vi "Turn.vi"(8 "Speed (0-30)":dbl=15.0, 11 "Angle (degrees)":i32=360) -> ()   [LabVIEW 2017]
uses:
  <vilib>/FPGAPlugInAG/myRIO-1900/niLvFpga_Open_myRIO-1900.vi
  <vilib>/rvi/interface/common/dynamic/niFpgaDynamicAddResources.vi
  <vilib>/Utility/error.llb/Error Cluster From Error Code.vi
  <vilib>/rvi/errors/niLvFpgaAdjustHostInterfaceError.vi
  <vilib>/FPGAPlugInAG/Dynamic/niLvFpga_Run_Dynamic.vi
  <vilib>/FPGAPlugInAG/Dynamic/niLvFpga_Close_Dynamic.vi
  <vilib>/rvi/interface/nirviOpenFPGA/nirviOpenFPGA.xnode
  FPGA Bitfiles/BadassLoader_FPGATarget_DCMotorControlle_4dRX-8eX8o0.lvbitx
  <vilib>/rvi/interface/nirviReadWriteControl/nirviReadWriteControl.xnode
  <vilib>/rvi/interface/nirviMethod/nirviMethod.xnode
  <vilib>/rvi/interface/nirviCloseFPGA/nirviCloseFPGA.xnode
  <vilib>/rvi/interface/Simulation/niFpgaSimulationCallBeginRW.vi
  NiFpgaLv.dll
panel:
  in  "stop":bool
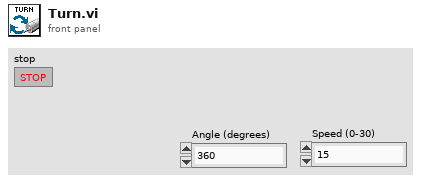
[diagram p1: front panel]
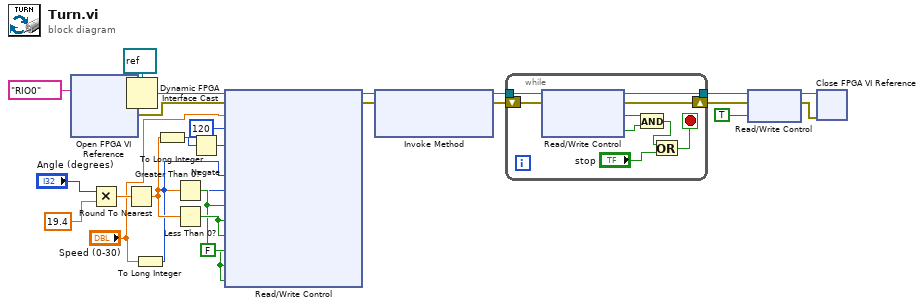
[diagram p0: block diagram]
diagram:
  w4 = FALSE ("stop")
  n1 = xnode "Open FPGA VI Reference"("resource name"=tag "RIO0") -> ("FPGA VI Reference Out"=w20:refnum<k20>, "error out"=w18:errorcluster)  [unwired: 1 in]
  n2 = Multiply(x="Angle (degrees)", y=19.4) -> (x*y=w22:dbl)
  n3 = Round To Nearest(number=w22) -> (nearest integer value=w16:dbl)
  n4 = Dynamic FPGA Interface Cast(Session In=refnum<k20> refnum ("FPGA Interface"), Type=w20) -> (Session Out=w19:refnum<k20>)
  n5 = To Long Integer(number="Speed (0-30)") -> (32bit integer=w2:i32)
  n6 = To Long Integer(number=w16) -> (32bit integer=w17:i32)
  n7 = Greater Than 0?(x=w16) -> (x > 0?=w6:bool)
  n8 = Less Than 0?(x=w16) -> (x < 0?=w7:bool)
  n9 = Negate(x=w17) -> (-x=w5:i32)
  n10 = xnode "Read/Write Control"("FPGA VI Reference In"=w19, "error in"=w18, "Slow velocity"="Speed (0-30)", "Ticks to slow"=120, "DCmotor_0_enc trgt"=w17, "DCmotor_1_enc trgt"=w5, "DCmotor_0_ccw vel sp"=w2, "DCmotor_1_ccw vel sp"=w2, "DCmotor_0_A"=w6, "DCmotor_0_B"=w7, "DCmotor_1_A"=w7, "DCmotor_1_B"=w6, "stop"=w4, "invert pulse (F)"=w4) -> ("FPGA VI Reference Out"=w13:refnum<k20>, "error out"=w12:errorcluster)
  n11 = xnode "Invoke Method"("FPGA VI Reference In"=w13, "error in"=w12) -> ("FPGA VI Reference Out"=w11:refnum<k20>, "error out"=w10:errorcluster)  [unwired: 1 in]
  n12 = while {
    tunnel: w11 -> [w35]
    tunnel: [w32] -> w15
    shift-right: [w30] -> w9
    shift-left: w10 -> [w31]
    stop <- w27 stop-if-true
    n13 = xnode "Read/Write Control"("FPGA VI Reference In"=w35, "error in"=w31) -> ("FPGA VI Reference Out"=w32:refnum<k20>, "error out"=w30:errorcluster, "M0_finished"=w34:bool, "M1_finished"=w33:bool)
    n14 = And(x=w34, y=w33) -> (x .and. y?=w29:bool)
    n15 = Or(x=w29, y="stop") -> (x .or. y?=w27:bool)
  }
  n16 = xnode "Read/Write Control"("FPGA VI Reference In"=w15, "error in"=w9, "stop"=TRUE) -> ("FPGA VI Reference Out"=w26:refnum<k20>, "error out"=w25:errorcluster)
  n17 = xnode "Close FPGA VI Reference"("FPGA VI Reference In"=w26, "error in"=w25) -> ()  [unwired: 1 out]
